vi "Common_UpdateAttributes.vi"(1 "ClassPath/LvClassRef":variant, 2 "NewAttributes":string, 3 "ClassInfo":T4[](array[typedef]), 5 "error in (no error)":errorcluster, 6 "Don't Prompt (False)":bool, 7 "Attributes":T1[](array[typedef]), 8 "Stereotype":string, 9 "Ctl-Description":string) -> (15 "CtlPath":path, 18 "Cancel":bool=TRUE, 19 "error out":errorcluster)   [LabVIEW 2020]
uses:
  CommonVIs_ClassNamePathType.ctl
  CommonVIs_AttributeType.ctl
  CommonVIs_AttributeDataType.ctl
  String/GDSString_AccessScopeModifierType.ctl
  Provider_BaseClassInterface/ClassReader_class/ClassReader.lvclass
panel:
  out "Path":path
  in  "Backup":bool
  out "New Attributes":string
  in  "Cancel":bool
  in  "OK":bool
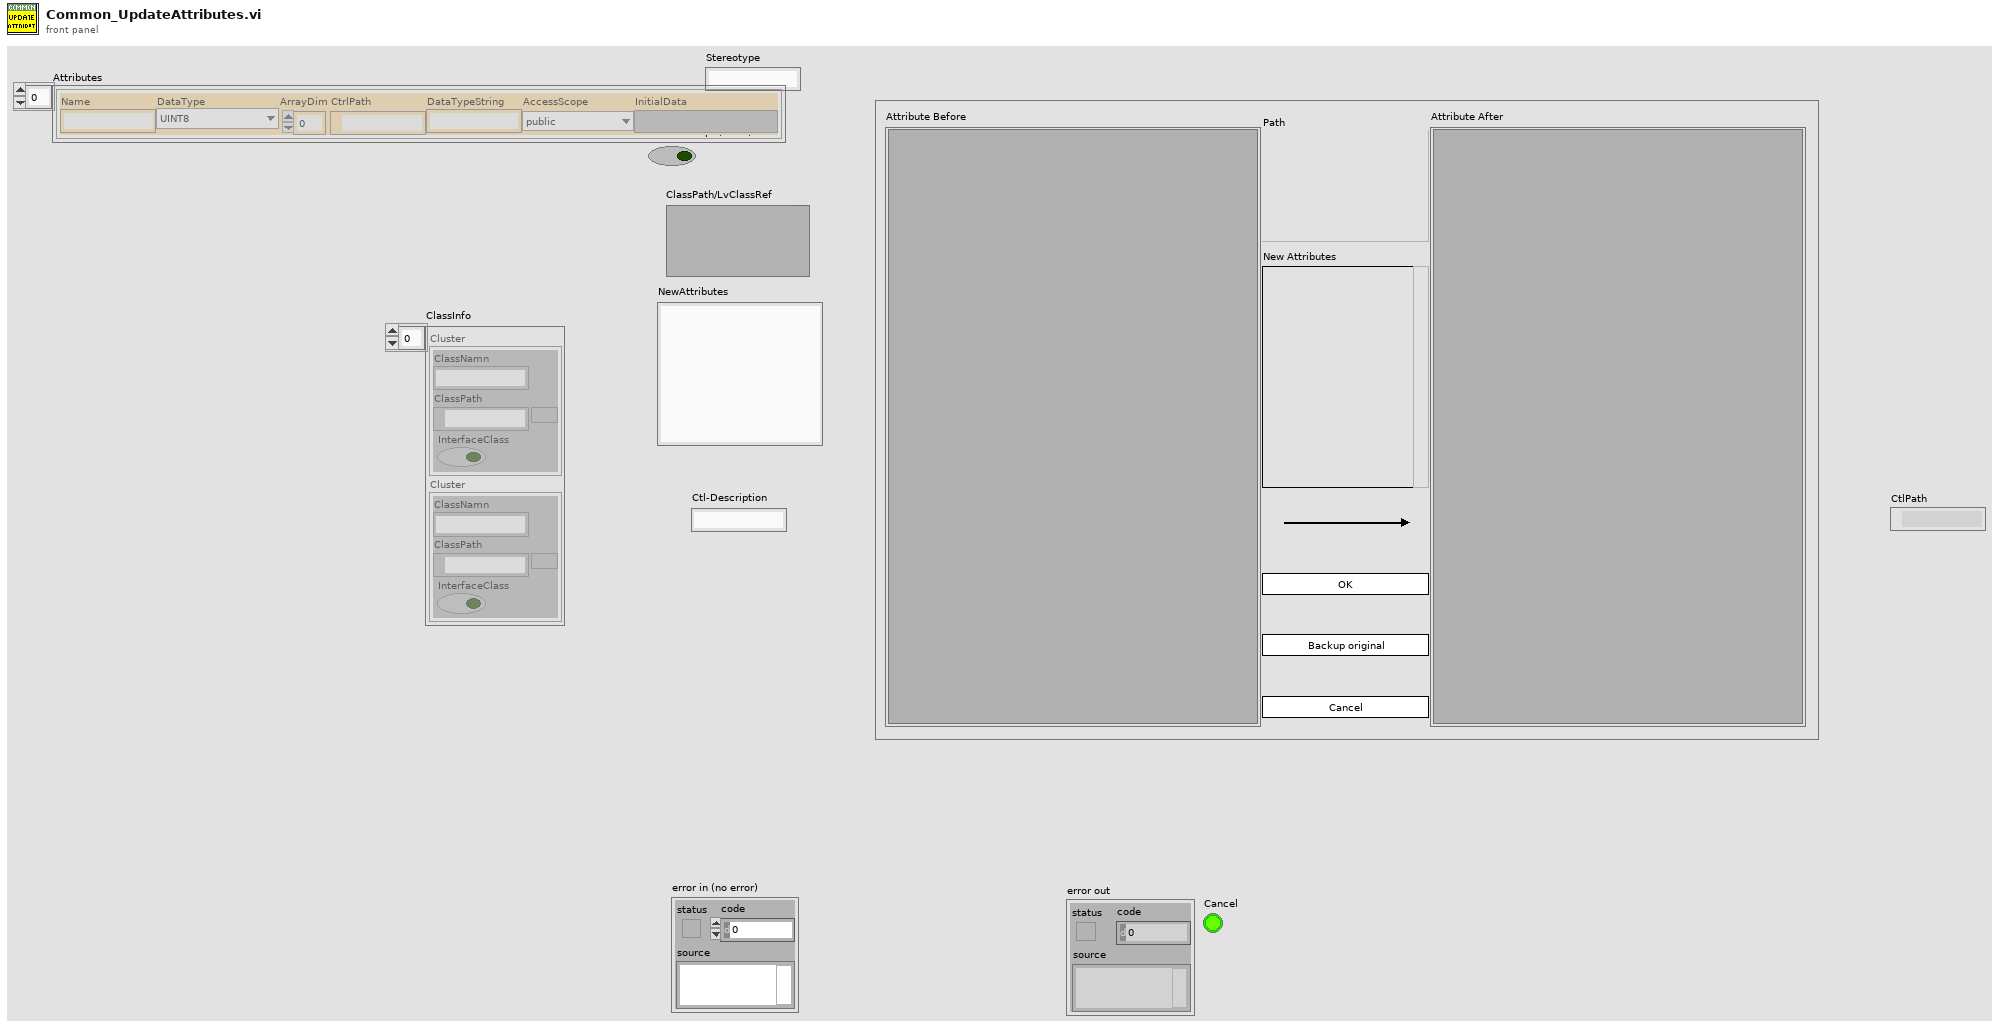
[diagram p1: front panel]
types:
  T1 = typedef "CommonVIs_AttributeType.ctl" = cluster{"Name":string, "DataType":T2, "ArrayDim":i32, "CtrlPath":path, "DataTypeString":string, "AccessScope":T3, "InitialData":variant}
  T2 = typedef "CommonVIs_AttributeDataType.ctl" = enum16{"UINT8", "INT8", "UINT16", "INT16", "UINT32", "INT32", "UINT64", "INT64", "SGL", "DBL", "EXT", "CSG", "CDB", "CXT", "TimeStamp", "STRING", "PATH", "BOOL", "ENUM", "RefNum", "VIRefNum", "LabVIEW Class", "Cluster", "Variant", "TypeDef", "Waveform", "LabVIEW Object", "Other", "void", "Set", "Map"}
  T3 = typedef "GDSString_AccessScopeModifierType.ctl" = enum16{"public", "private", "protected", "internal"}
  T4 = typedef "CommonVIs_ClassNamePathType.ctl" = cluster{"ClassNamn":string, "ClassPath":path, "InterfaceClass":bool}
  T5 = cluster{"OrgCtrl":refnum<vi>, "TemplateControl":path, "NewCtrl":refnum<vi>, "NewCluster":refnum<vi>, "BaseCtrl":refnum<vi>, "AddedCtrls":refnum<vi>[], "Cancel":bool, "Attributes":T1[], "BaseClassType":i16[], "OrgCluster":refnum<vi>, "OrgClusterMembers":cluster{"name":string, "AttributeDataType":T2, "Dims":i16}[], "OrgClusterCtrls":refnum<vi>[], "ClassVi":refnum<vi>, "WaveformControl":path, "EnumControl":path, "Enum":bool, "NewEnum":refnum<vi>, "OrgEnum":refnum<vi>, "ClusterCanBeEmpty":bool, "NewControlCreated":bool, "NoUpdate":bool, "AutoUpdate":bool, "CtlPath":path}
  T6 = enum32{"invalid VI type", "Standard VI", "Control VI", "Global VI", "Polymorphic VI", "Configuration VI"}
  T7 = enum32{"Extended Precision", "Double Precision", "Single Precision", "Long", "Word", "Byte", "Unsigned Long", "Unsigned Word", "Unsigned Byte", "Complex Extended", "Complex Double", "Complex Single", "Quad", "Unsigned Quad"}
  T8 = enum32{"Invalid", "Standard", "Closed", "Hidden", "Minimized", "Maximized"}
  T9 = typedef "CommonVIs_AttributeInfoType.ctl" = cluster{"name":string, "type":T2, "dimension":i32, "typeName":string, "typePath":path, "visibility":T10}
  T10 = typedef "CommonVIs_VisibilityType.ctl" = enum16{"Public", "Private", "Protected"}
  T11 = cluster{"name":string, "AttributeDataType":T2, "Dims":i16}[]
  T12 = cluster{"name":string, "AttributeDataType":T2, "Dims":i16}
  T13 = typedef "LVPointTypeDef.ctl" = cluster{"Horizontal":i16, "Vertical":i16}
  T14 = enum32{"existing file", "new file", "new or existing file", "existing dir", "new dir", "new or existing dir", "existing file (use LLBs)", "new file (use LLBs)", "new or existing file (use LLBs)", "new or existing file or directory (use LLBs)"}
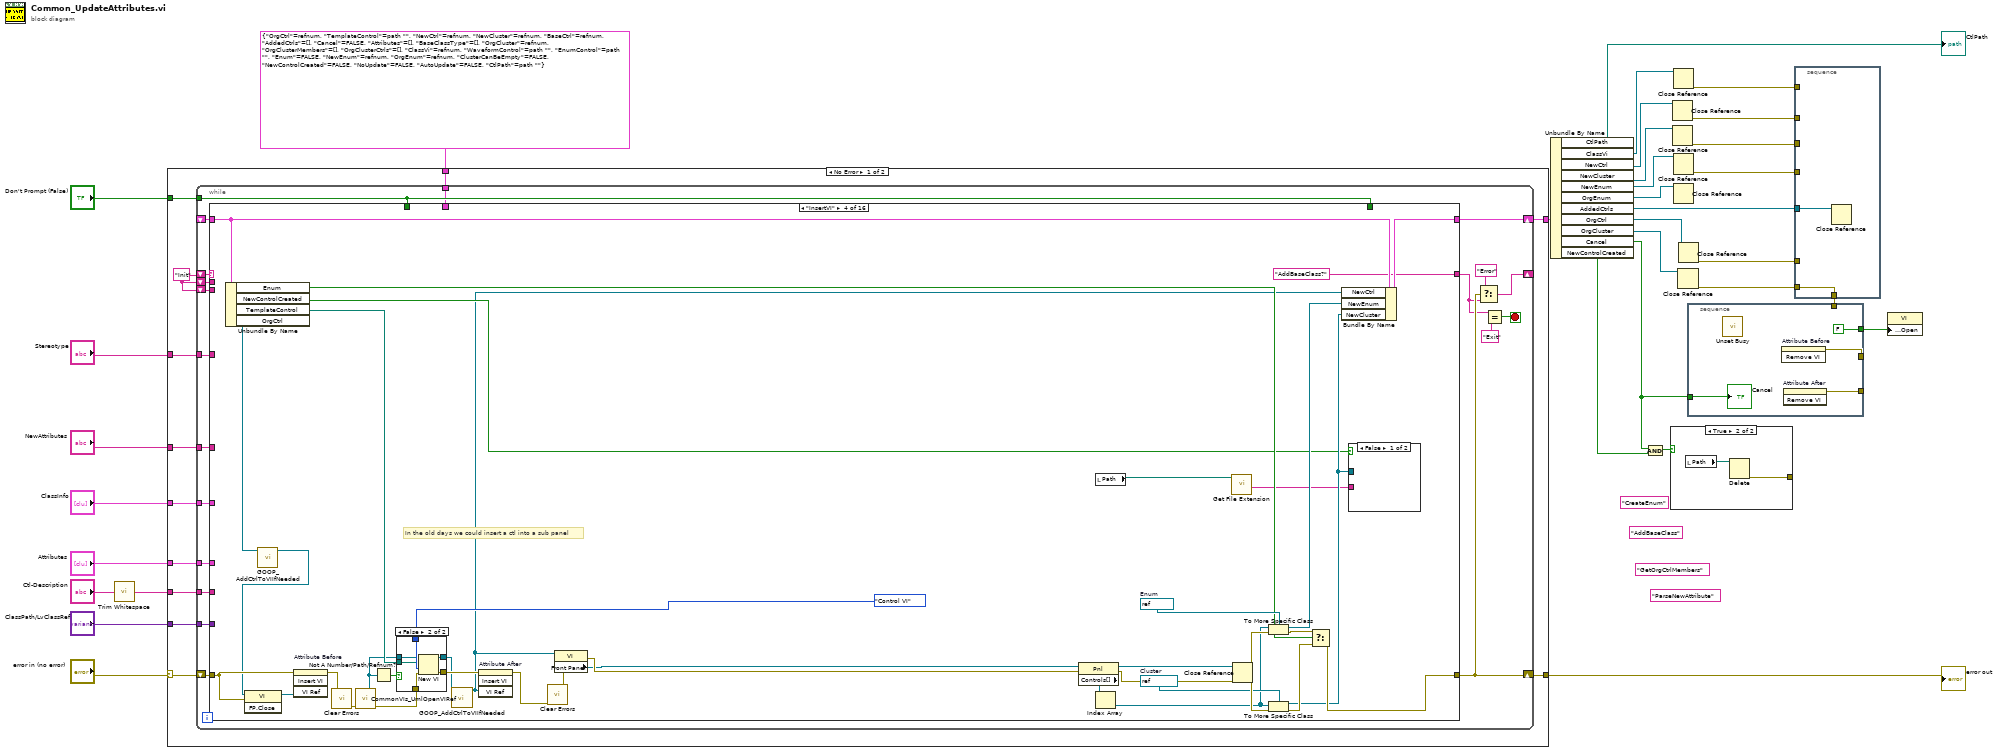
[diagram p0: block diagram]
diagram:
  (unwired) "ParseNewAttribute" ("y")
  (unwired) "GetOrgCtrlMembers" ("y")
  (unwired) "AddBaseClass" ("y")
  (unwired) "CreateEnum" ("y")
  n1 = call <vilib>:"Trim Whitespace.vi"("string"="Ctl-Description") -> ("trimmed string"=w2:string)  [unwired: 1 in]
  n2 = case shown="No Error" "error in (no error)" {
    selector: "error in (no error)" -> [w44 w1117]
    tunnel: [w43 w1117] -> w31
    tunnel: "ClassPath/LvClassRef" -> [w42 _]
    tunnel: [w41 _] -> w22
    tunnel: "NewAttributes" -> [w40 _]
    tunnel: "ClassInfo" -> [w39 _]
    tunnel: "Don't Prompt (False)" -> [w38 _]
    tunnel: "Stereotype" -> [w37 _]
    tunnel: T5 {"OrgCtrl"=refnum, "TemplateControl"=path "", "NewCtrl"=refnum, "NewCluster"=refnum, "BaseCtrl"=refnum, "AddedCtrls"=[], "Cancel"=FALSE, "Attributes"=[], "BaseClassType"=[], "OrgCluster"=refnum, "OrgClusterMembers"=[], "OrgClusterCtrls"=[], "ClassVi"=refnum, "WaveformControl"=path "", "EnumControl"=path "", "Enum"=FALSE, "NewEnum"=refnum, "OrgEnum"=refnum, "ClusterCanBeEmpty"=FALSE, "NewControlCreated"=FALSE, "NoUpdate"=FALSE, "AutoUpdate"=FALSE, "CtlPath"=path ""} -> [w35 _]
    tunnel: "Attributes" -> [w34 _]
    tunnel: w2 -> [w33 _]
    frame No Error {
      w36 = "Init"
      n3 = while {
        shift-right: [w63] -> w43
        shift-left: w44 -> [w64]
        shift-right: [w57] -> _
        shift-left: w36 -> [w62]
        tunnel: w42 -> [w61]
        shift-right: [w60] -> w41
        shift-left: _ -> [w59]
        tunnel: w40 -> [w53]
        tunnel: w39 -> [w52]
        tunnel: w38 -> [w50]
        shift-left: w36 -> [w51]
        tunnel: w37 -> [w49]
        shift-left: w36 -> [w48]
        tunnel: w35 -> [w47]
        tunnel: w34 -> [w46]
        tunnel: w33 -> [w45]
        stop <- w54 stop-if-true
        n4 = case shown="\"InsertVI\"" w62 {
          tunnel: w64 -> [w72 w130 w208 w268 w302 w364 w392 w428 w453 w474 w506 w857 w877 w940 w1014 w1059]
          tunnel: w61 -> [_ w100 _ _ _ _ _ _ _ _ _ _ _ _ _ _]
          tunnel: [w66 w92 "Init" "AddBaseClass?" w301 "Move Controls" ("y") "GetOrgCtrlMembers" ("y") "ParseNewAttribute" ("y") "None?" ("y") "AddControls" ("y") "Move Controls" ("y") w849 w873 "ReplaceCtrl" ("y") "AddToProject?" ("y") "Exit" ("y")] -> w56
          tunnel: [w70 w128 w202 w259 w298 w359 w381 w425 w450 w466 w503 w845 w872 w935 w949 w1056] -> w60
          tunnel: [w71 w129 w205 w272 w304 w363 w393 w430 w453 w474 w505 w857 w877 w937 w994 w1058] -> w63
          tunnel: w59 -> [w70 _ w202 w262 w293 w359 w382 w423 w451 w464 w491 w845 w870 w935 w981 w1056]
          tunnel: w53 -> [_ w118 _ _ _ w361 _ _ w449 _ _ _ _ _ _ _]
          tunnel: w52 -> [_ _ _ _ _ _ _ _ w439 _ w481 _ _ _ _ _]
          tunnel: w50 -> [_ _ _ _ _ _ _ _ _ _ _ w848 _ _ _ _]
          tunnel: w51 -> [w69 _ _ _ _ _ _ _ _ _ _ _ _ _ _ _]
          tunnel: w50 -> [_ _ _ _ _ _ _ _ _ w465 _ _ _ _ _ _]
          tunnel: w49 -> [_ w107 _ _ _ _ _ _ _ _ _ _ _ _ _ _]
          tunnel: w48 -> [w65 _ _ _ _ _ _ _ _ _ _ _ _ _ _ _]
          tunnel: w47 -> [_ w91 _ _ _ _ _ _ _ _ _ _ _ _ _ _]
          tunnel: w46 -> [_ _ _ _ _ w356 _ _ w442 _ _ _ _ _ _ _]
          tunnel: w45 -> [_ _ _ _ _ _ _ _ _ _ _ _ _ _ w950 _]
          frame "Error", Default {
            n5 = Unbundle By Name(w72) -> ("source"=w68:string, "code"=w67:i32)
            n6 = case shown="0, Default" w67 {
              tunnel: w69 -> [_ w85]
              tunnel: w68 -> [_ _]
              tunnel: w72 -> [w78 _]
              tunnel: [w77 errorcluster {"status"=FALSE, "code"=0, "source"=""}] -> w71
              tunnel: ["Exit" ("y") w87] -> w66
              tunnel: w65 -> [w74 _]
              frame 0, Default {
                n7 = Equal?(x=w74, y="Error" ("t")) -> (x = y?=w73:bool)
                n8 = Select(t=errorcluster {"status"=FALSE, "code"=0, "source"=""}, s=w73, f=w78) -> (s? t:f=w77:errorcluster)
              }
              frame 1073 {
                n9 = call "CommonVIs_TwoButtonDialog.vi"("message"="The object attribute file is currently being used by other VIs.\nPlease stop the execution of the VIs that uses this object attributes.", "yesButtonName"="Retry" ("T button name (\"OK\")"), "noButtonName"="Cancel" ("F button name (\"Cancel\")"), "WindowTitle"="Warning") -> ("yesButtonPressed"=w80:bool)  [unwired: 2 in, 13 out]
                n10 = Select(t=w85, s=w80, f="Exit" ("y")) -> (s? t:f=w87:string)
              }
            }
          }
          frame "Init" {
            n11 = Variant To Data(type=path path "", Variant=w100) -> (data=w98:path)  [unwired: 1 in, 1 out]
            n12 = Current VI's Path() -> (path=w126:path)
            n13 = call <vilib>:"Get File Extension.vi"("file"=w98) -> ("lowercase file extension"=w99:string)  [unwired: 1 in, 9 out]
            n14 = Strip Path(path=w126) -> (stripped path=w111:path, name=w125:string)
            n15 = case shown="Default" w99 {
              tunnel: w130 -> [w171 w190]
              tunnel: [w171 w189] -> w129
              tunnel: [w169 w173] -> w97
              tunnel: w100 -> [_ w180]
              tunnel: [w170 w172] -> w94
              tunnel: w98 -> [w170 _]
              tunnel: [_ w176] -> w96
              tunnel: [_ w187] -> _
              tunnel: [_ w186] -> _
              frame "ctl" {
                n16 = call "CommonVIs_UmlOpenVIRef.vi"("error in"=w171, "ViPath/ViName"=w170) -> ("vi reference"=w169:refnum<vi>)  [unwired: 2 in, 7 out]
              }
              frame Default {
                n17 = call "CreateReaderFromClass.vi"("ClassPath/LvClassRef"=w180, "error in"=w190) -> ("ClassReader"=w185:refnum<class "ClassReader.lvclass">, "error out"=w192:errorcluster)  [unwired: 16 out]
                n18 = Variant To Data(type=refnum<vi> refnum ("LVClass.Open"), Variant=w180) -> (error out=w188:errorcluster)  [unwired: 1 in, 1 out]
                n19 = call-dynamic "GetAttributes.vi"("ClassReader in"=w185, "OnlyGetReference"=TRUE, "error in (no error)"=w192) -> ("ClassReader out"=w183:refnum<class "ClassReader.lvclass">, "ObjectAttributeReference"=w174:refnum<vi>, "ClassAttributeReference"=w182:refnum<vi>, "error out"=w191:errorcluster)  [unwired: 13 out]
                n20 = Close Reference(reference=w182) -> (error out=w187:errorcluster)  [unwired: 1 in]
                n21 = case shown="No Error" w188 {
                  tunnel: w183 -> [w193 w196]
                  tunnel: w191 -> [w194 w198]
                  tunnel: [w194 w197] -> w189
                  tunnel: [w193 w195] -> w175
                  frame No Error {
                  }
                  frame Error {
                    n22 = call-dynamic "CleanUp.vi"("reference in"=w196, "error in (no error)"=w198) -> ("reference out"=w195:refnum<class "ClassReader.lvclass">, "error out"=w197:errorcluster)  [unwired: 16 out]
                  }
                }
                n23 = Flatten To String(anything=w175) -> (data string=w177:string)  [unwired: 1 in, 4 out]
                n24 = Match Pattern(string=w177, regular expression="ClassReaderNative") -> (offset past match=w179:i32)  [unwired: 4 out]
                n25 = property class="VI"(reference=w174) -> (reference out=w173:refnum<vi>, error out=w186:errorcluster, "Path"=w172:path)  [unwired: 1 in]
                n26 = Greater Or Equal To 0?(x=w179) -> (x >= 0?=w176:bool)
              }
            }
            "Path" <- w94
            n27 = String Length(string=w125) -> (length=w124:i32)
            n28 = Subtract(x=w124, y=19) -> (x-y=w122:i32)
            n29 = case shown="False" FALSE {
              tunnel: [_ w131] -> w90
              frame False {
              }
              frame True {
                n30 = property class="App"() -> ("App.VersionYear"=w134:string)  [unwired: 2 in, 2 out]
                n31 = Decimal String To Number(string=w134) -> (number=w133:i32)  [unwired: 2 in, 1 out]
                n32 = Greater Or Equal?(x=w133, y=2013) -> (x >= y?=w131:bool)
              }
            }
            n33 = To Upper Case(1:w107) -> (0:w105:string)
            n34 = String Subset(string=w125, offset (0)=0, length (rest)=w122) -> (substring=w113:string)
            n35 = Concatenate Strings(w113, "TemplateObjectAttributes.ctt" ("string")) -> (w120:string)
            n36 = Concatenate Strings(w113, "TemplateWaveform.ctt" ("string")) -> (w114:string)
            n37 = Concatenate Strings(w113, "TemplateEnum.ctt" ("string")) -> (w110:string)
            n38 = Empty String/Path?(string/path=w94) -> (empty?=w93:bool)
            n39 = Build Path(base path=w111, name or relative path=w120) -> (appended path=w109:path)
            n40 = Build Path(base path=w111, name or relative path=w114) -> (appended path=w115:path)
            n41 = Build Path(base path=w111, name or relative path=w110) -> (appended path=w108:path)
            n42 = Match Pattern(string=w105, regular expression="ENUM") -> (offset past match=w104:i32)  [unwired: 4 out]
            n43 = Greater Or Equal To 0?(x=w104) -> (x >= 0?=w103:bool)
            n44 = Select(t=w108, s=w103, f=w109) -> (s? t:f=w102:path)
            n45 = case shown="False" w93 {
              tunnel: [w142 _] -> w127
              tunnel: [w141 _] -> w117
              tunnel: w102 -> [w140 _]
              tunnel: w94 -> [w138 _]
              tunnel: w97 -> [w137 _]
              tunnel: [w136 _] -> w95
              tunnel: ["InsertVI" ("Left Button Text (\"Yes\")") "Exit" ("y")] -> w92
              frame False {
                n46 = Not A Number/Path/Refnum?(number/path/refnum=w137) -> (NaN/Path/Refnum?=w139:bool)
                n47 = case shown="False" w139 {
                  tunnel: [w159 w165] -> w142
                  tunnel: w137 -> [w159 _]
                  tunnel: w140 -> [_ w164]
                  tunnel: [w143 _] -> w141
                  tunnel: w138 -> [w145 w163]
                  tunnel: [_ TRUE] -> w136
                  tunnel: [_ w167] -> _
                  frame False {
                    n48 = Strip Path(path=w145) -> (stripped path=w155:path)  [unwired: 1 out]
                    n49 = Strip Path(path=w155) -> (stripped path=w152:path)  [unwired: 1 out]
                    n50 = List Folder(path=w155, pattern="*Create.vi" ("FileSearchPattern")) -> (filenames=w158:string[])  [unwired: 1 in, 4 out]
                    n51 = List Folder(path=w152, pattern="*Create.vi" ("FileSearchPattern")) -> (path out=w150:path, filenames=w151:string[])  [unwired: 1 in, 3 out]
                    n52 = Array Size(array=w158) -> (size(s)=w157:i32)
                    n53 = Index Array(array=w158) -> (element=w154:string)  [unwired: 1 in]
                    n54 = Index Array(array=w151) -> (element=w149:string)  [unwired: 1 in]
                    n55 = Equal To 0?(x=w157) -> (x = 0?=w148:bool)
                    n56 = Build Path(base path=w155, name or relative path=w154) -> (appended path=w146:path)
                    n57 = Build Path(base path=w150, name or relative path=w149) -> (appended path=w147:path)
                    n58 = Select(t=w147, s=w148, f=w146) -> (s? t:f=w144:path)
                    n59 = call "CommonVIs_UmlOpenVIRef.vi"("ViPath/ViName"=w144) -> ("vi reference"=w143:refnum<vi>)  [unwired: 3 in, 7 out]
                  }
                  frame True {
                    # "CREATE FILE"
                    n60 = call <vilib>:"Librarian Copy.vi"("source"=w164, "destination"=w163) -> ("dup destination"=w162:path)  [unwired: 3 in, 6 out]
                    n61 = Set Permissions(7:i16 511 ("permissions"), 11:w162) -> (3:w161:path)  [unwired: 3 in, 1 out]
                    n62 = call "CommonVIs_UmlOpenVIRef.vi"("ViPath/ViName"=w161) -> ("error out"=w167:errorcluster, "vi reference"=w165:refnum<vi>)  [unwired: 3 in, 6 out]
                  }
                }
              }
              frame True {
              }
            }
            n63 = Bundle By Name(cluster=w91, "AutoUpdate"=w90, "Enum"=w103, "TemplateControl"=w102, "WaveformControl"=w115, "EnumControl"=w108, "ClusterCanBeEmpty"=w96, "NewControlCreated"=w95, "ClassVi"=w117, "OrgCtrl"=w127) -> (w128:T5)
            "New Attributes" <- w118
          }
          frame "AutoCloseAll" {
            n64 = Unbundle By Name(w202) -> ("OrgCtrl"=w201:refnum<vi>)
            n65 = property class="VI"(reference=w201) -> ("Callers' Names"=w204:string[])  [unwired: 1 in, 2 out]
            n66 = while {
              shift-right: [w218] -> _
              shift-left: w204 -> [w219]
              shift-right: [w222] -> w207
              shift-left: w208 -> [w223]
              shift-right: [w216] -> w200
              shift-left: refnum<vi>[] [] -> [w217]
              stop <- w220 stop-if-true
              n67 = Array Size(array=w219) -> (size(s)=w221:i32)
              n68 = case shown="Default" w221 {
                tunnel: [w227 TRUE] -> w220
                tunnel: w219 -> [w234 w239]
                tunnel: w223 -> [w236 w241]
                tunnel: [w228 w239] -> w218
                tunnel: [w235 w241] -> w222
                tunnel: w217 -> [w226 w238]
                tunnel: [w224 w238] -> w216
                frame Default {
                  n69 = Delete From Array(array=w234, index=0) -> (deleted portion=w232:string, array with subset deleted=w230:string[])  [unwired: 1 in]
                  n70 = Open VI Reference(vi path=w232, error in (no error)=w236) -> (vi reference=w231:refnum<vi>, error out=w237:errorcluster)  [unwired: 4 out]
                  n71 = property class="VI"(reference=w231, error in=w237) -> (reference out=w225:refnum<vi>, error out=w235:errorcluster, "Callers' Names"=w229:string[])
                  n72 = Unbundle By Name(w235) -> ("status"=w227:bool)
                  n73 = Build Array (concatenate)(w230, w229) -> (w228:string[])
                  n74 = Build Array (concatenate)(w226, w225) -> (w224:refnum<vi>[])
                }
                frame 0 {
                }
              }
            }
            n75 = for {
              shift-right: [w214] -> w206
              shift-left: w207 -> [w213]
              tunnel: w200 -> [w209] mode=indexing
              n76 = invoke class="VI" method="Abort VI"(reference=w209, error in=w213) -> (reference out=w211:refnum<vi>)  [unwired: 1 in, 2 out]
              n77 = property class="VI"(reference=w211, error in=w213, "Front Panel Window:Open"=FALSE) -> (reference out=w210:refnum<vi>, error out=w215:errorcluster)
              n78 = Close Reference(reference=w210, error in (no error)=w215) -> (error out=w214:errorcluster)
            }
            n79 = Close Reference(reference=w201, error in (no error)=w206) -> (error out=w205:errorcluster)
          }
          frame "InsertVI" {
            w257 = refnum<vi> refnum  # Enum
            w260 = refnum<vi> refnum  # Cluster
            # "In the old days we could insert a ctl into a sub panel"
            n80 = Unbundle By Name(w262) -> ("Enum"=w255:bool, "NewControlCreated"=w251:bool, "TemplateControl"=w253:path, "OrgCtrl"=w245:refnum<vi>)
            n81 = call "GOOP_AddCtrlToVIIfNeeded.vi"("Ctrl VI in"=w245) -> ("VI out"=w244:refnum<vi>)  [unwired: 8 in, 2 out]
            n82 = invoke class="VI" method="FP.Close"(reference=w244, error in=w268) -> (reference out=w248:refnum<vi>)  [unwired: 1 in, 2 out]
            n83 = invoke on="Attribute Before" class="SubPanel" method="Insert VI"(error in=w268, "VI Ref"=w248) -> (error out=w271:errorcluster)  [unwired: 2 in, 3 out]
            n84 = call <vilib>:"Clear Errors.vi"("error in (no error)"=w271) -> ("error out"=w267:errorcluster)  [unwired: 5 in, 1 out]
            n85 = call "CommonVIs_UmlOpenVIRef.vi"("error in"=w267) -> ("error out"=w270:errorcluster, "AppRefOut"=w247:refnum<vi>)  [unwired: 3 in, 6 out]
            n86 = Not A Number/Path/Refnum?(number/path/refnum=w247) -> (NaN/Path/Refnum?=w246:bool)
            n87 = case shown="False" w246 {
              tunnel: T6."Control VI" ("vi type (standard vi)") -> [w281 w287]
              tunnel: [w280 w286] -> w243
              tunnel: w270 -> [w283 w289]
              tunnel: [w282 w288] -> w269
              tunnel: w253 -> [w279 w285]
              tunnel: w247 -> [_ w284]
              frame True {
                n88 = New VI(8:w283, 9:w281, 10:w279) -> (0:w282:errorcluster, 3:w280:refnum<vi>)  [unwired: 4 out]
              }
              frame False {
                n89 = New VI(8:w289, 9:w287, 10:w285, 11:w284) -> (0:w288:errorcluster, 3:w286:refnum<vi>)  [unwired: 3 out]
              }
            }
            n90 = call "GOOP_AddCtrlToVIIfNeeded.vi"("Ctrl VI in"=w243) -> ("VI out"=w242:refnum<vi>)  [unwired: 8 in, 2 out]
            n91 = invoke on="Attribute After" class="SubPanel" method="Insert VI"(error in=w269, "VI Ref"=w242) -> (error out=w278:errorcluster)  [unwired: 2 in, 3 out]
            n92 = call <vilib>:"Clear Errors.vi"("error in (no error)"=w278) -> ("error out"=w266:errorcluster)  [unwired: 5 in, 1 out]
            n93 = property class="VI"(reference=w242, error in=w266) -> (error out=w276:errorcluster, "Front Panel"=w264:refnum<vi>)  [unwired: 1 out]
            n94 = property class="Pnl"(reference=w264, error in=w276) -> (reference out=w261:refnum<vi>, error out=w277:errorcluster, "Controls[]"=w263:refnum<vi>[])
            n95 = local read "Path"() -> (w250:path)
            n96 = Index Array(array=w263) -> (element=w256:refnum<vi>)  [unwired: 1 in]
            n97 = call <vilib>:"Get File Extension.vi"("file"=w250) -> ("filename without extension"=w249:string)  [unwired: 1 in, 9 out]
            n98 = Close Reference(reference=w261, error in (no error)=w277) -> (error out=w275:errorcluster)
            n99 = To More Specific Class(target class=w257, reference=w256, error in=w275) -> (specific class reference=w254:refnum<vi>, error out=w274:errorcluster)
            n100 = To More Specific Class(target class=w260, reference=w256, error in=w275) -> (specific class reference=w252:refnum<vi>, error out=w273:errorcluster)
            n101 = Select(t=w274, s=w255, f=w273) -> (s? t:f=w272:errorcluster)
            n102 = Bundle By Name(cluster=w262, "NewCtrl"=w242, "NewEnum"=w254, "NewCluster"=w252) -> (w259:T5)
            n103 = case shown="False" w251 {
              tunnel: w252 -> [_ w291]
              tunnel: w249 -> [_ w290]
              frame False {
              }
              frame True {
                n104 = property class="Clust"(reference=w291, "Label.Text"=w290) -> ()  [unwired: 1 in, 2 out]
              }
            }
          }
          frame "AddBaseClass?" {
            w300 = refnum<vi> refnum  # Cluster
            n105 = Unbundle By Name(w293) -> ("Enum"=w292:bool)
            n106 = Unbundle By Name(w293) -> ("OrgCtrl"=w296:refnum<vi>)
            n107 = property class="VI"(reference=w296, error in=w302) -> (error out=w306:errorcluster, "Front Panel"=w295:refnum<vi>)  [unwired: 1 out]
            n108 = property class="Pnl"(reference=w295, error in=w306) -> (error out=w305:errorcluster, "Controls[]"=w299:refnum<vi>[])  [unwired: 1 out]
            n109 = Index Array(array=w299) -> (element=w294:refnum<vi>)  [unwired: 1 in]
            n110 = To More Specific Class(target class=w300, reference=w294, error in=w305) -> (specific class reference=w297:refnum<vi>, error out=w303:errorcluster)
            n111 = case shown="No Error" w303 {
              tunnel: [w309 w343] -> w301
              tunnel: w303 -> [w320 _]
              tunnel: w293 -> [w317 w340]
              tunnel: [w316 w339] -> w298
              tunnel: [w322 w345] -> w304
              tunnel: w297 -> [w314 _]
              tunnel: w302 -> [_ w345]
              tunnel: w294 -> [_ w342]
              tunnel: w292 -> [w307 w337]
              frame No Error {
                # "Base Class Type"
                # "BaseClass Found"
                n112 = property class="Clust"(reference=w314, error in=w320) -> (error out=w321:errorcluster, "Controls[]"=w312:refnum<vi>[])  [unwired: 1 out]
                n113 = for {
                  N: 1 -> [_]
                  tunnel: w320 -> [w333]
                  tunnel: [w327] -> w311
                  tunnel: [w325] -> w315
                  tunnel: w312 -> [w323] mode=indexing
                  w324 = "Base class" ("x")
                  n114 = property class="Ctl"(reference=w323, error in=w333) -> ("Label.Text"=w330:string, "Class Name"=w332:string, "Type Descriptor"=w326:i16[])  [unwired: 2 out]
                  n115 = Equal?(x=w332, y="Cluster") -> (x = y?=w328:bool)
                  n116 = Equal?(x=w324, y=w330) -> (x = y?=w329:bool)
                  n117 = And(x=w329, y=w328) -> (x .and. y?=w327:bool)
                  n118 = call "CommonVIs_TypeDescNonNameDepentent.vi"("Type DescriptorNameDependent"=w326, "LabelText"=w324) -> ("Type DescriptorNonNameDependent"=w325:i16[])  [unwired: 17 out]
                }
                n119 = for {
                  shift-right: [w335] -> w322
                  shift-left: w321 -> [w336]
                  tunnel: w312 -> [w334] mode=indexing
                  tunnel: w311 -> [_]
                  n120 = Close Reference(reference=w334, error in (no error)=w336) -> (error out=w335:errorcluster)
                }
                n121 = Bundle By Name(cluster=w317, "OrgCluster"=w314, "BaseClassType"=w315) -> (w316:T5)
                n122 = Select(t="AddBaseClass" ("y"), s=w311, f="GetOrgCtrlMembers" ("y")) -> (s? t:f=w310:string)
                n123 = Select(t="CreateEnum" ("y"), s=w307, f=w310) -> (s? t:f=w309:string)
              }
              frame Error {
                w341 = refnum<vi> refnum  # Enum
                n124 = To More Specific Class(target class=w341, reference=w342) -> (specific class reference=w338:refnum<vi>, error out=w344:errorcluster)  [unwired: 1 in]
                n125 = case shown="No Error" w344 {
                  tunnel: [w347 "Exit" ("y")] -> w343
                  tunnel: w340 -> [w352 w353]
                  tunnel: [w351 w353] -> w339
                  tunnel: w338 -> [w350 _]
                  tunnel: w337 -> [w349 _]
                  frame No Error {
                    n126 = Select(t="CreateEnum" ("y"), s=w349, f="ParseNewAttribute" ("y")) -> (s? t:f=w347:string)
                    n127 = Bundle By Name(cluster=w352, "OrgEnum"=w350) -> (w351:T5)
                  }
                  frame Error {
                    n128 = One Button Dialog(message="Only cluster controls are supported") -> ()  [unwired: 2 out]
                  }
                }
              }
            }
          }
          frame "CreateEnum" {
            n129 = Empty Array?(array=w356) -> (empty?=w357:bool)
            n130 = Unbundle By Name(w359) -> ("NewEnum"=w362:refnum<vi>)
            n131 = case shown="False" w357 {
              tunnel: w361 -> [_ w374]
              tunnel: [w365 w369] -> w360
              tunnel: w356 -> [w366 _]
              frame False {
                n132 = for {
                  tunnel: w366 -> [w368] mode=indexing
                  tunnel: [w367] -> w365 mode=indexing
                  n133 = Unbundle By Name(w368) -> ("Name"=w367:string)
                }
              }
              frame True {
                n134 = call <vilib>:"Trim Whitespace.vi"("string"=w374) -> ("trimmed string"=w373:string)  [unwired: 1 in]
                n135 = Spreadsheet String To Array(delimiter (Tab)="\n", format string="%s", spreadsheet string=w373, array type (2D Dbl)=string[] []) -> (array=w369:string[])
              }
            }
            n136 = property class="Enum"(reference=w362, error in=w364, "Strings []"=w360) -> (error out=w363:errorcluster)  [unwired: 1 out]
          }
          frame "AddBaseClass" {
            w387 = refnum<vi> refnum  # Cluster
            w388 = 21607 items=[".NET Refnum", "Absolute Value", "Access Rights", "ActiveX Container", "Add", "Add Array Elements", "Agitator", "AllSpoll", "And", "And Array Elements", "Append True/False String", "Application Refnum", "Array", "Array 1", "Array Constant", "Array Max & Min", "Array Size", "Array Subset", "Array To Cluster", "Array To Spreadsheet String", "Array of Strings to Path", "Atmospheric Tank", "Atmospheric Tank 1", "Automation Close", "Automation Open", "Automation Refnum", "Avogadro Constant (1/mol)", "Base 10 Logarithm Of e", "Bin", "Bin 1", "Bluetooth Close Connection", "Bluetooth Create Listener", "Bluetooth Discover", "Bluetooth Network Connection Refnum", "Bluetooth Open Connection", "Bluetooth Read", "Bluetooth Wait On Listener", "Bluetooth Write", "Boolean Array To Number", "Boolean To (0,1)", "Build Array", "Build Cluster Array", "Build Path", "Build Waveform", "Bundle", "Bundle By Name", "Byte Array To String", "Byte Stream File Refnum", "Call By Reference Node", "Call Chain", "Call Library Function Node", "Cancel Button", "Cancel Button 1", "Cancel Notification", "Carriage Return Constant", "Case Structure", "Cast Unit Bases", "Check Valve", "Checkbox", "Class Specifier Constant", "Classic Radio Buttons", "Close File", "Close Reference", "Cluster", "Cluster 1", "Cluster Constant", "Cluster To Array", "Code Interface Node", "Color Box", "Color Box Constant", "Color Box Thin Border", "Color Ramp", "Combo Box", "Combo Box 1", "Combo Box Constant", "Complex Conjugate", "Complex To Polar", "Complex To Re/Im", "Compound Arithmetic", "Compressor", "Concatenate Strings", "Conditional Disable Structure", "Constructor Node", "Control Help Window", "Control Online Help", "Control Refnum", "Convert Unit", "Conveyer", "Copy", "Cosecant", "Cosine", "Cotangent", "Create User Event", "Current VI's Menubar", "Current VI's Path", "DAQmx Analog Trigger Source", "DAQmx Analog Trigger Source 1", "DAQmx Analog Trigger Source 2", "DAQmx Analog Trigger Source Constant", "DAQmx Device Name", "DAQmx Device Name 1", "DAQmx Device Name 2", "DAQmx Device Name Constant", "DAQmx Global Channel", "DAQmx Global Channel 1", "DAQmx Global Channel 2", "DAQmx Global Channel Constant", "DAQmx Physical Channel", "DAQmx Physical Channel 1", "DAQmx Physical Channel 2", "DAQmx Physical Channel Constant", "DAQmx Scale Name", "DAQmx Scale Name 1", "DAQmx Scale Name 2", "DAQmx Scale Name Constant", "DAQmx Switch", "DAQmx Switch 1", "DAQmx Switch 2", "DAQmx Switch Constant", "DAQmx Task Name", "DAQmx Task Name 1", "DAQmx Task Name 2", "DAQmx Task Name Constant", "DAQmx Terminal", "DAQmx Terminal 1", "DAQmx Terminal 2", "DAQmx Terminal Constant", "Data Log File Refnum", "DataSocket Close", "DataSocket Open", "DataSocket Read", "DataSocket Refnum", "DataSocket Write", "Database Variant To Data", "Date/Time To Seconds", "Decimal Digit?", "Decimal String To Number", "Decimate 1D Array", "Decrement", "Default Directory", "Delete", "Delete From Array", "Delete Menu Items", "Delete Variant Attribute", "Delete Waveform Attribute", "Dequeue Element", "Destroy User Event", "DevClear", "DevClearList", "Device Control/Status", "Device Refnum", "Diagram Disable Structure", "Dial", "Dial 1", "Dialog Button", "Dialog Checkbox", "Dialog Chiseled Line", "Dialog Colored Rectangle", "Dialog Combo Box", "Dialog Horizontal Pointer Slide", "Dialog Horizontal Progress Bar", "Dialog Horizontal Slide", "Dialog Label", "Dialog Listbox", "Dialog Listbox 1", "Dialog Multicolumn Listbox", "Dialog Multiple Selection Multicolumn Listbox", "Dialog Numeric", "Dialog Path Control", "Dialog Pict Ring", "Dialog Radio Button", "Dialog Radio Buttons", "Dialog Recessed Frame", "Dialog Ring", "Dialog Spin Control", "Dialog String", "Dialog Tab Control", "Dialog Table", "Dialog Tree", "Dialog Vertical Pointer Slide", "Dialog Vertical Progress Bar", "Dialog Vertical Slide", "Digital Data", "Digital Data 1", "Digital Waveform Graph", "Digital Waveform Graph 1", "Digital Waveform Graph 2", "Divide", "Dlg CheckBox", "Dlg Horiz Scrollbar", "Dlg Numeric", "Dlg Numeric 2", "Dlg String", "Dlg Vert Scrollbar", "Down Arrow", "Down Bow Valve", "Down Bow Valve 1", "Down Bow Valve 2", "Down Rect Valve", "Down Rect Valve 1", "Down Rect Valve 2", "Down Tee", "Down Tee 1", "EOF", "Elementary Charge (C)", "Empty Path Constant", "Empty String Constant", "Empty String/Path?", "Enable Menu Tracking", "EnableLocal", "EnableRemote", "End of Line Constant", "Enqueue Element", "Enqueue Element At Opposite End", "Enum", "Enum 1", "Enum Constant", "Equal To 0?", "Equal?", "Error Ring Constant", "Event Callback Refnum", "Event Structure", "Exchanger", "Exclusive Or", "Exponential", "Exponential (Arg) -1", "Expression Node", "False Constant", "Feedback Node", "FieldPoint IO Point", "FieldPoint IO Point 1", "FieldPoint IO Point Constant", "File Dialog", "File Path Control", "File Path Control 1", "File Path Indicator", "File Path Indicator 1", "File/Directory Info", "FindLstn", "FindRQS", "First Call?", "Flat Box", "Flat Circle", "Flat Down Triangle", "Flat Frame", "Flat Left Triangle", "Flat Right Triangle", "Flat Round Button", "Flat Rounded Box", "Flat Sequence Structure", "Flat Square Button", "Flat Up Triangle", "Flatten To String", "Flatten To XML", "Flattened String To Variant", "Flush File", "Flush Queue", "For Loop", "Format Date/Time String", "Format Into File", "Format Into String", "Format Value", "Formula Node", "Fract/Exp String To Number", "Framed Color Box", "Framed Color Box 1", "Free Label", "Furnace", "GPIB Clear", "GPIB Initialization", "GPIB Misc", "GPIB Read", "GPIB Serial Poll", "GPIB Status", "GPIB Trigger", "GPIB Wait", "GPIB Write", "Gauge", "Gauge 1", "Generate Front Panel Activity", "Generate Occurrence", "Generate User Event", "Generic Refnum", "Generic Refnum By Reference Flatten", "Generic Refnum Deep Copy", "Generic Refnum Name", "Generic Refnum Tag", "Generic Refnum Tag By Reference Flatten", "Generic Refnum Tag Flatten", "Get Date/Time In Seconds", "Get Date/Time String", "Get Help Window Status", "Get Menu Item Info", "Get Menu Selection", "Get Menu Short Cut Info", "Get Notifier Status", "Get Queue Status", "Get Variant Attribute", "Get Waveform Attribute", "Get Waveform Components", "Global Variable", "Gravitational Constant (N m2/kg2)", "Greater Or Equal To 0?", "Greater Or Equal?", "Greater Than 0?", "Greater?", "Handle Peek", "Handle Poke", "Hex Digit?", "Hexadecimal String To Number", "HiQ-Script", "Hopper", "Hopper 1", "Horiz Line", "Horiz Pipe", "Horiz Pipe 1", "Horizontal Button Box", "Horizontal Fill Slide", "Horizontal Fill Slide 1", "Horizontal Graduated Bar", "Horizontal Pointer Slide", "Horizontal Pointer Slide 1", "Horizontal Progress Bar", "Horizontal Slide", "Horizontal Slide Switch", "Horizontal Smooth Box", "Horizontal Switch", "Horizontal Tank", "Horizontal Toggle Switch", "Horizontal Toggle Switch 1", "Hyperbolic Cosine", "Hyperbolic Sine", "Hyperbolic Tangent", "IMAQ Session", "IP To String", "IVI Delete Session", "IVI Logical Name", "IVI Logical Name 1", "IVI Logical Name Constant", "IVI New Session", "Implies", "In Range and Coerce", "Increment", "Index & Bundle Cluster Array", "Index Array", "Index String Array", "Initialize Array", "Insert Into Array", "Insert Menu Items", "Intensity Chart", "Intensity Chart 1", "Intensity Graph", "Intensity Graph 1", "Interleave 1D Arrays", "Interpolate 1D Array", "Inverse Cosine", "Inverse Hyperbolic Cosine", "Inverse Hyperbolic Sine", "Inverse Hyperbolic Tangent", "Inverse Sine", "Inverse Tangent", "Inverse Tangent (2 Input)", "Invoke Node", "IrDA Close Connection", "IrDA Create Listener", "IrDA Discover", "IrDA Network Connection Refnum", "IrDA Open Connection", "IrDA Read", "IrDA Wait On Listener", "IrDA Write", "Join Numbers", "Knob", "Knob 1", "LED Button", "Label", "Labeled Oblong Button", "Labeled Rectangular Button", "Labeled Round Button", "Labeled Square Button", "Left Arrow", "Left Bow Valve", "Left Bow Valve 1", "Left Bow Valve 2", "Left Down Elbow", "Left Down Elbow 1", "Left Pump", "Left Pump 1", "Left Rect Valve", "Left Rect Valve 1", "Left Rect Valve 2", "Left Tee", "Left Tee 1", "Left Up Elbow", "Left Up Elbow 1", "Less Or Equal To 0?", "Less Or Equal?", "Less Than 0?", "Less?", "Lexical Class", "Line Feed Constant", "List Directory", "Listbox", "Listbox 1", "Listbox Symbol Ring Constant", "Local Variable", "Lock Range", "Logarithm Base 10", "Logarithm Base 2", "Logarithm Base X", "Logical Shift", "Lowered Rounded Box", "MATLAB Script", "MakeAddr", "Mantissa & Exponent", "Match First String", "Match Pattern", "Match True/False String", "Max & Min", "Menu Refnum", "Menu Ring", "Menu Ring 1", "Menu-Popup Ring", "Merge Signals", "Meter", "Meter 1", "Molar Gas Constant (J/(mol K))", "Motion Resource", "Motion Resource 1", "Motion Resource Constant", "Motor", "Motor 1", "Move", "Multicolumn Listbox", "Multicolumn Listbox 1", "Multicolumn Listbox 2", "Multicolumn Listbox 3", "Multicolumn Listbox 4", "Multiple Selection Listbox", "Multiple Selection Listbox 1", "Multiple Selection Listbox 2", "Multiple Selection Listbox 3", "Multiple Selection Multicolumn Listbox", "Multiply", "Multiply Array Elements", "Natural Logarithm", "Natural Logarithm (Arg +1)", "Natural Logarithm Base", "Natural Logarithm Of 10", "Natural Logarithm Of 2", "Natural Logarithm Of Pi", "Negate", "Negative Infinity", "New Directory", "New File", "New VI", "New VI Object", "Not", "Not A Number/Path/Refnum?", "Not A Path Constant", "Not And", "Not Equal To 0?", "Not Equal?", "Not Exclusive Or", "Not Or", "Not a Refnum Constant", "Not a Tag", "Number To Boolean Array", "Number To Decimal String", "Number To Engineering String", "Number To Exponential String", "Number To Fractional String", "Number To Hexadecimal String", "Number To Octal String", "Numeric Constant", "Numeric Control", "Numeric Control 1", "Numeric Indicator", "Numeric Indicator 1", "OK Button", "OLE Variant", "Obtain Notifier", "Obtain Queue", "Occurrence Refnum", "Octal Digit?", "Octal String To Number", "Old VISA Open", "One Button Dialog", "Open Application Reference", "Open Device", "Open File", "Open File (New)", "Open Tank", "Open Tank 1", "Open VI Object Reference", "Open VI Reference", "Or", "Or Array Elements", "PPoll", "PPollConfig", "PPollUnconfig", "PassControl", "Path Constant", "Path To String", "Path Type", "Path to Array of Strings", "Pi", "Pi Divided By 2", "Pi Multiplied By 2", "Pick Line", "Pict Ring", "Pict Ring 1", "Picture", "PixMap", "PixMap (Do not touch it!!)", "Planck Constant (J/Hz)", "Platform Flat Square Button", "Plug-In Control", "Polar To Complex", "Positive Infinity", "Power Of 10", "Power Of 2", "Power Of X", "Pressure Tank", "Pressure Tank 1", "Preview Queue Element", "Printable?", "Property Node", "Pulldown Menu Ring", "Push Button", "Quit LabVIEW", "Quotient & Remainder", "Radio Buttons", "Raised Box", "Raised Box 1", "Raised Circle", "Raised Down Triangle", "Raised Frame", "Raised Left Triangle", "Raised Right Triangle", "Raised Rounded Box", "Raised Up Triangle", "Random Number (0-1)", "RcvRespMsg", "Re/Im To Complex", "Read Binary File", "Read Device", "Read File", "ReadStatus", "Receive", "ReceiveSetup", "Recessed Box", "Recessed Circle", "Recessed Down Triangle", "Recessed Frame", "Recessed Left Triangle", "Recessed Menu Ring", "Recessed Right Triangle", "Recessed Rounded Box", "Recessed Up Triangle", "Reciprocal", "Reciprocal Of Pi", "Reciprocal Of e", "Rectangular Stop Button", "Refnum to Path", "Refnum to Session", "Register Event Callback", "Register For Events", "Register Session", "Release Notifier", "Release Queue", "Replace Array Subset", "Replace Substring", "Request Deallocation", "ResetSys", "Reshape Array", "Reverse 1D Array", "Reverse String", "Right Arrow", "Right Bow Valve", "Right Bow Valve 1", "Right Bow Valve 2", "Right Down Elbow", "Right Down Elbow 1", "Right Pump", "Right Pump 1", "Right Rect Valve", "Right Rect Valve 1", "Right Rect Valve 2", "Right Tee", "Right Tee 1", "Right Up Elbow", "Right Up Elbow 1", "Ring Constant", "Rocker", "Rotary Feeder", "Rotate", "Rotate 1D Array", "Rotate Left With Carry", "Rotate Right With Carry", "Rotate String", "Round Button", "Round LED", "Round LED 1", "Round Light", "Round Push Button", "Round Push Button 2", "Round Radio Button", "Round Stop Button", "Round To +Infinity", "Round To -Infinity", "Round To Nearest", "Rydberg Constant (/m)", "Scale By Power Of 2", "Scan From File", "Scan From String", "Scan String For Tokens", "Scan Value", "Search 1D Array", "Search and Replace String", "Search/Split String", "Secant", "Seconds To Date/Time", "Seek", "Select", "Send", "Send Notification", "SendCmds", "SendDataBytes", "SendIFC", "SendLLO", "SendList", "SendSetup", "Session to Refnum", "Set Menu Item Info", "Set Occurrence", "Set Variant Attribute", "Set Waveform Attribute", "SetRWLS", "SetTimeOut", "Sign", "Simple Horizontal Slide", "Simple Numeric", "Simple Numeric 1", "Simple String", "Simple Vertical Slide", "Simulation Loop", "Sinc", "Sine", "Sine & Cosine", "Single Selection Listbox", "Size Handle", "Slide Switch", "Sort 1D Array", "Speed Of Light In Vacuum (m/sec)", "Split 1D Array", "Split Button", "Split Number", "Split Signals", "Spreadsheet String To Array", "Square Button", "Square LED", "Square LED 1", "Square Light", "Square Push Button", "Square Push Button 2", "Square Radio Button", "Square Root", "Stacked Sequence Structure", "Standard ListBox", "State Diagram", "Static VI Reference", "Stop", "Stop Button", "String Constant", "String Control", "String Control 1", "String Indicator", "String Indicator 1", "String Length", "String Subset", "String To Byte Array", "String To IP", "String To Path", "String to Tag", "Strip Path", "SubPanel", "SubPanel (Classic)", "Subtract", "Swap Bytes", "Swap Vector Element", "Swap Words", "TCP Close Connection", "TCP Create Listener", "TCP Flattened Read", "TCP Flattened Write", "TCP Flex Read", "TCP Flex Write", "TCP Network Connection Refnum", "TCP Open Connection", "TCP Read", "TCP Wait On Listener", "TCP Write", "Tab Constant", "Tab Control", "Tab Control 1", "Table", "Table 1", "Table 2", "Tag Attribute Ring", "Tag Constant", "Tag Control", "Tag Control 1", "Tag Indicator", "Tag Indicator 1", "Tag to String", "Tangent", "Tank", "Tank 1", "Temporary Directory", "TestSRQ", "TestSys", "Text & Pict Ring", "Text & Pict Ring 1", "Text Button", "Text Ring", "Text Ring 1", "Thermometer", "Thermometer 1", "Thick Chiseled Line", "Thick Line", "Thick Line with Arrow", "Thick Lowered Box", "Thin Chiseled Line", "Thin Line", "Thin Line with Arrow", "Threshold 1D Array", "Tick Count (ms)", "Time Stamp Constant", "Time Stamp Control", "Time Stamp Control 1", "Time Stamp Indicator", "Time Stamp Indicator 1", "Timed Loop", "To Byte Integer", "To Double Precision Complex", "To Double Precision Float", "To Extended Precision Complex", "To Extended Precision Float", "To Long Integer", "To Lower Case", "To More Generic Class", "To More Specific Class", "To OLE Variant", "To Quad Integer", "To Single Precision Complex", "To Single Precision Float", "To Time Stamp", "To Unsigned Byte Integer", "To Unsigned Long Integer", "To Unsigned Quad Integer", "To Unsigned Word Integer", "To Upper Case", "To Variant", "To Word Integer", "Traditional DAQ Channel", "Traditional DAQ Channel 1", "Traditional DAQ Channel Constant", "Transpose 2D Array", "Tree", "Trigger", "TriggerList", "Two Button Dialog", "Type Cast", "Type and Creator", "UDP Close", "UDP Multicast Open", "UDP Network Connection Refnum", "UDP Open", "UDP Read", "UDP Write", "Unbundle", "Unbundle By Name", "Unflatten From String", "Unflatten From XML", "Uniform Dbl Waveform", "Uniform Int16 Waveform", "Unregister For Events", "Unregister Session", "Up Arrow", "Up Bow Valve", "Up Bow Valve 1", "Up Bow Valve 2", "Up Rect Valve", "Up Rect Valve 1", "Up Rect Valve 2", "Up Tee", "Up Tee 1", "User Item", "VI Library", "VI Refnum", "VISA Assert Interrupt Signal", "VISA Assert Trigger", "VISA Assert Utility Signal", "VISA Clear", "VISA Close", "VISA Disable Event", "VISA Discard Events", "VISA Enable Event", "VISA Find Resource", "VISA Flush I/O Buffer", "VISA GPIB Command", "VISA GPIB Control ATN", "VISA GPIB Control REN", "VISA GPIB Pass Control", "VISA GPIB Send IFC", "VISA In 16", "VISA In 32", "VISA In 8", "VISA Lock", "VISA Map Address", "VISA Map Trigger", "VISA Memory Allocation", "VISA Memory Free", "VISA Move", "VISA Move In 16", "VISA Move In 32", "VISA Move In 8", "VISA Move Out 16", "VISA Move Out 32", "VISA Move Out 8", "VISA Open", "VISA Out 16", "VISA Out 32", "VISA Out 8", "VISA Peek 16", "VISA Peek 32", "VISA Peek 8", "VISA Poke 16", "VISA Poke 32", "VISA Poke 8", "VISA Read", "VISA Read STB", "VISA Read To File", "VISA Refnum to Session", "VISA Resource Name", "VISA Resource Name Constant", "VISA Set I/O Buffer Size", "VISA Status Description", "VISA USB Control In", "VISA USB Control Out", "VISA Unlock", "VISA Unmap Address", "VISA Unmap Trigger", "VISA VXI Cmd or Query", "VISA Wait on Event", "VISA Write", "VISA Write From File", "VISA resource name", "Variant", "Variant To Data", "Variant To Flattened String", "Vert Line", "Vert Pipe", "Vert Pipe 1", "Vert Rocker", "Vertical Fill Slide", "Vertical Fill Slide 1", "Vertical Graduated Bar", "Vertical Pointer Slide", "Vertical Pointer Slide 1", "Vertical Progress Bar", "Vertical Slide", "Vertical Slide Switch", "Vertical Slide Switch 1", "Vertical Smooth Box", "Vertical Switch", "Vertical Toggle Switch", "Vertical Toggle Switch 1", "Volume Info", "Wait (ms)", "Wait For Activity", "Wait For Front Panel Activity", "Wait Until Next ms Multiple", "Wait for GPIB RQS", "Wait on Notification", "Wait on Notification from Multiple", "Wait on Occurrence", "WaitSRQ", "Waveform Chart", "Waveform Chart 1", "Waveform Chart 2", "Waveform Graph", "Waveform Graph 1", "While Loop", "While Loop 1", "White Space?", "Write Device", "Write File", "XY Graph", "XY Graph 1", "Xmath Script"]
            n137 = Unbundle By Name(w382) -> ("BaseClassType"=w375:i16[], "OrgCtrl"=w378:refnum<vi>)
            n138 = property class="VI"(reference=w378, error in=w392) -> ("Callees' Names"=w377:string[])  [unwired: 2 out]
            n139 = Array Size(array=w377) -> (size(s)=w376:i32)
            n140 = while {
              tunnel: [w410] -> w385
              tunnel: w377 -> [w396] mode=indexing
              tunnel: [w413] -> w391
              tunnel: w376 -> [w407]
              tunnel: w375 -> [w399]
              i -> [w408]
              stop <- w406 stop-if-true
              n141 = call "CommonVIs_UmlOpenVIRef.vi"("ViPath/ViName"=w396) -> ("error out"=w412:errorcluster, "vi reference"=w395:refnum<vi>)  [unwired: 3 in, 6 out]
              n142 = Increment(x=w408) -> (x+1=w409:i32)
              n143 = Greater Or Equal?(x=w409, y=w407) -> (x >= y?=w397:bool)
              n144 = property class="VI"(reference=w395, error in=w412) -> (reference out=w411:refnum<vi>, error out=w414:errorcluster, "VI Path"=w410:path, "Front Panel"=w405:refnum<vi>)
              n145 = property class="Pnl"(reference=w405) -> ("Controls[]"=w404:refnum<vi>[])  [unwired: 1 in, 2 out]
              n146 = Index Array(array=w404) -> (element=w403:refnum<vi>)  [unwired: 1 in]
              n147 = property class="Ctl"(reference=w403) -> ("Type Descriptor"=w402:i16[], "Label.Text"=w401:string)  [unwired: 1 in, 2 out]
              n148 = Close Reference(reference=w411, error in (no error)=w414) -> (error out=w413:errorcluster)
              n149 = call "CommonVIs_TypeDescNonNameDepentent.vi"("Type DescriptorNameDependent"=w402, "LabelText"=w401) -> ("Type DescriptorNonNameDependent"=w400:i16[])  [unwired: 17 out]
              n150 = Equal?(x=w399, y=w400) -> (x = y?=w398:bool)
              n151 = Or(x=w397, y=w398) -> (x .or. y?=w406:bool)
            }
            n152 = Unbundle By Name(w382) -> ("NewCluster"=w386:refnum<vi>)
            n153 = New VI Object(vi object class=w387, owner refnum=w386, style=w388, position/next to=cluster{"Horizontal":i16, "Vertical":i16} {"Horizontal"=0, "Vertical"=0}, 6:w385, 8:w391) -> (object refnum=w389:refnum<vi>, 0:w394:errorcluster)  [unwired: 2 out]
            n154 = property class="Clust"(reference=w389, error in=w394, "Label.Visible"=TRUE) -> (reference out=w380:refnum<vi>, error out=w393:errorcluster)
            n155 = Build Array(w380) -> (w379:refnum<vi>[])
            n156 = Bundle By Name(cluster=w382, "AddedCtrls"=w379) -> (w381:T5)
          }
          frame "GetOrgCtrlMembers" {
            (unwired) CommonVIs_AttributeDataType."UINT8" ("AttributeDataType")
            (unwired) CommonVIs_AttributeDataType."UINT8" ("type")
            n157 = Unbundle By Name(w423) -> ("OrgCluster"=w424:refnum<vi>)
            n158 = property class="Clust"(reference=w424, error in=w428) -> (error out=w429:errorcluster, "Controls[]"=w421:refnum<vi>[])  [unwired: 1 out]
            n159 = call "Common_GetClassAttrubutes.vi"("CtlRefnum"=w424, "error in (no error)"=w429) -> ("attributeInfo"=w426:T9[], "error out"=w430:errorcluster)  [unwired: 2 in, 14 out]
            n160 = Unbundle By Name(w423) -> ("AddedCtrls"=w422:refnum<vi>[], "OrgClusterMembers"=w416:T11)
            n161 = Array Size(array=w422) -> (size(s)=w418:i32)
            n162 = Index Array(array=w416) -> (element=w415:T12)  [unwired: 1 in]
            n163 = for {
              tunnel: w426 -> [w438] mode=indexing
              tunnel: [w436] -> w417 mode=indexing
              tunnel: w415 -> [w432]
              n164 = Unbundle By Name(w438) -> ("name"=w437:string, "dimension"=w434:i32, "type"=w433:T2)
              n165 = To Word Integer(number=w434) -> (16bit integer=w431:i16)
              n166 = To Lower Case(string=w437) -> (all lower case string=w435:string)
              n167 = Bundle(cluster=w432, "name"=w435, "AttributeDataType"=w433, "Dims"=w431) -> (w436:T12)
            }
            n168 = Delete From Array(array=w421, length=w418, index=0) -> (array with subset deleted=w420:refnum<vi>[])  [unwired: 1 out]
            n169 = Bundle By Name(cluster=w423, "OrgClusterCtrls"=w420, "OrgClusterMembers"=w417) -> (w425:T5)
          }
          frame "ParseNewAttribute" {
            n170 = call <vilib>:"Trim Whitespace.vi"("string"=w449) -> ("trimmed string"=w446:string)  [unwired: 1 in]
            n171 = Empty Array?(array=w442) -> (empty?=w443:bool)
            n172 = Spreadsheet String To Array(delimiter (Tab)="\n", format string="%s", spreadsheet string=w446, array type (2D Dbl)=string[] []) -> (array=w444:string[])
            n173 = case shown="True" w443 {
              tunnel: w444 -> [_ w460]
              tunnel: [w457 w459] -> w441
              tunnel: w439 -> [_ w458]
              tunnel: w442 -> [w457 _]
              frame False {
              }
              frame True {
                n174 = call "CommonVIs_AttributeToDataType.vi"("ClassInfo"=w458, "Array"=w460) -> ("Attributes"=w459:T1[])
              }
            }
            n175 = for {
              tunnel: w441 -> [w456] mode=indexing
              tunnel: [w455] -> w440 mode=indexing
              tunnel: w439 -> [w454]
              n176 = call "CommonVIs_UpdateAttributeCtrlPath.vi"("ClassInfo"=w454, "DataType in"=w456) -> ("DataType out"=w455:T1)  [unwired: 9 in]
            }
            n177 = Bundle By Name(cluster=w451, "Attributes"=w440) -> (w450:T5)
          }
          frame "None?" {
            n178 = Unbundle By Name(w464) -> ("AddedCtrls"=w471:refnum<vi>[], "Attributes"=w472:T1[])
            n179 = Array Size(array=w471) -> (size(s)=w470:i32)
            n180 = Array Size(array=w472) -> (size(s)=w469:i32)
            n181 = Equal To 0?(x=w470) -> (x = 0?=w468:bool)
            n182 = Equal To 0?(x=w469) -> (x = 0?=w467:bool)
            n183 = Compound Arithmetic op=AND(w468, w467, invert FALSE ("value")) -> (w462:bool)
